vi "Create Build Array.vi"   [LabVIEW 2012, in "Scripting Tools.lvlib"]
uses:
  Scripting Tools.lvlib
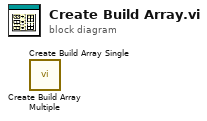
[diagram p0: block diagram]
diagram:
  n1 = call "Create Build Array Multiple.vi"() -> ()  [unwired: 9 in, 3 out]
  n2 = call "Create Build Array Single.vi"() -> ()  [unwired: 9 in, 3 out]
